vi "term_create_constant.vi"() -> ()   [LabVIEW 2022 SP3]
panel:
  out "Create Constant":refnum<vi>
  out "error out":errorcluster
  out "reference out":refnum<vi>
  in  "Value":variant
  in  "error in (no error)":errorcluster
  in  "reference":refnum<vi>
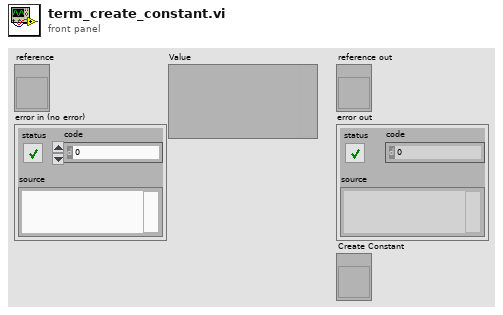
[diagram p1: front panel]
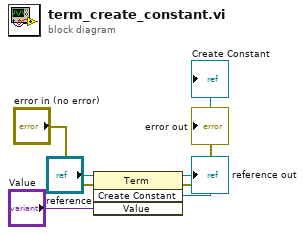
[diagram p0: block diagram]
diagram:
  n1 = invoke class="Term" method="Create Constant"(reference="reference", error in="error in (no error)", "Value"="Value") -> (reference out=→"reference out":refnum<vi>, error out=→"error out":errorcluster, "Create Constant"=→"Create Constant":refnum<vi>)  [unwired: 1 in, 1 out]
